vi "Stimulus.Open.vi"(8 "error in (no error)":errorcluster, 11 "State Variables":T1={"Events.State"=refnum, "Events.Test Result"=refnum, "Events.Progress"=refnum, "INI.Settings"={"Build Location"=path "C:/Simple Sequence Editor/SequenceRepo", "LoggingLocation"=path "", "Sequence.AbortChannel"="", "Sequence.IterationInfoChannel"="", "Sequence.DurationChannel"="", "Sequence.StepInfoChannel"="", "Sequence.SkipChannel"="", "PlotChannels"=[], "Sequence.InitializeScript"=path "C:/Simple Sequence Editor/SequenceRepo", "Sequence.CleanupScript"=path "", "Log.DefaultRate"=0.0}, "NIVS.AlarmManager"=refnum, "NIVS.BaseLogPath"=path "", "NIVS.DataLogManagerRef"=refnum, "NIVS.DataLogSpecRef"=refnum, "NIVS.Deployed"=FALSE, "NIVS.Events"={"SequenceEvent"=refnum, "SystemChangeEvent"=refnum, "WorkspaceEvent"=refnum}, "NIVS.GatewayIPAddress"="", "NIVS.DataLogGUID"="", "NIVS.ProfileCallback"=refnum, "NIVS.ProfileRef"=refnum, "NIVS.SequenceState"=enum."Idle", "NIVS.SystemDefinitionFile"=path "", "NIVS.SystemStateRefs"={"CustDatRef"=refnum, "EvtRef"=refnum, "Target State User Event"=refnum}, "NIVS.WorkspaceManager"=refnum, "NIVS.EventLogGUID"="", "NIVS.EventLogManagerRef"=refnum, "NIVS.EventLogSpecRef"=refnum, "NIVS.BaseToolPath"=path "", "Restart.Path"=path "", "Sequence.#ofColumns"=0, "Sequence.Iterations"=0, "Sequence.Channels"=[], "Sequence.ValidConfig?"=FALSE, "Station.ID"="", "UDP.Queue"=refnum, "UI.Abort"=refnum, "UI.Alarms"=refnum, "UI.Apply"=refnum, "UI.Back"=refnum, "UI.BaseFileName"=refnum, "UI.CurrentIteration"=refnum, "UI.CurrentStep"=refnum, "UI.CyclicFrequency"=refnum, "UI.Description"=refnum, "UI.DelayTime"=refnum, "UI.DisableAlarms"=refnum, "UI.Duration"=refnum, "UI.EnableLogging"=refnum, "UI.EnableState"=refnum, "UI.High"=refnum, "UI.LogChannels"=refnum, "UI.Low"=refnum, "UI.MonitoredVariable"=refnum, "UI.Next"=refnum, "UI.NumberOfCycles"=refnum, "UI.OperatorName"=refnum, "UI.Pause"=refnum, "UI.Profile"=refnum, "UI.Revert"=refnum, "UI.Skip"=refnum, "UI.Start"=refnum, "UI.StartIteration"=refnum, "UI.StartStep"=refnum, "UI.TabControl"=refnum, "UI.TotalIterations"=refnum, "UI.WaveformDefinition"=refnum, "UI.WaveformPreview"=refnum, "UI.WorkOrderNumber"=refnum, "UI.Chart"=refnum, "UI.Status"=refnum, "UI.DataView"=refnum, "UI.Table"=refnum, "UI.Multihead"=refnum, "UI.ToolTab"=refnum, "UI.Result"=refnum, "UI.Log Path"=refnum, "UI.ReportPath"=refnum, "UI.RestartPath"=refnum, "UI.AlarmLog"=refnum}) -> (0 "error out":errorcluster, 3 "State Variables":T1={"Events.State"=refnum, "Events.Test Result"=refnum, "Events.Progress"=refnum, "INI.Settings"={"Build Location"=path "C:/Simple Sequence Editor/SequenceRepo", "LoggingLocation"=path "", "Sequence.AbortChannel"="", "Sequence.IterationInfoChannel"="", "Sequence.DurationChannel"="", "Sequence.StepInfoChannel"="", "Sequence.SkipChannel"="", "PlotChannels"=[], "Sequence.InitializeScript"=path "C:/Simple Sequence Editor/SequenceRepo", "Sequence.CleanupScript"=path "", "Log.DefaultRate"=0.0}, "NIVS.AlarmManager"=refnum, "NIVS.BaseLogPath"=path "", "NIVS.DataLogManagerRef"=refnum, "NIVS.DataLogSpecRef"=refnum, "NIVS.Deployed"=FALSE, "NIVS.Events"={"SequenceEvent"=refnum, "SystemChangeEvent"=refnum, "WorkspaceEvent"=refnum}, "NIVS.GatewayIPAddress"="", "NIVS.DataLogGUID"="", "NIVS.ProfileCallback"=refnum, "NIVS.ProfileRef"=refnum, "NIVS.SequenceState"=enum."Idle", "NIVS.SystemDefinitionFile"=path "", "NIVS.SystemStateRefs"={"CustDatRef"=refnum, "EvtRef"=refnum, "Target State User Event"=refnum}, "NIVS.WorkspaceManager"=refnum, "NIVS.EventLogGUID"="", "NIVS.EventLogManagerRef"=refnum, "NIVS.EventLogSpecRef"=refnum, "NIVS.BaseToolPath"=path "", "Restart.Path"=path "", "Sequence.#ofColumns"=0, "Sequence.Iterations"=0, "Sequence.Channels"=[], "Sequence.ValidConfig?"=FALSE, "Station.ID"="", "UDP.Queue"=refnum, "UI.Abort"=refnum, "UI.Alarms"=refnum, "UI.Apply"=refnum, "UI.Back"=refnum, "UI.BaseFileName"=refnum, "UI.CurrentIteration"=refnum, "UI.CurrentStep"=refnum, "UI.CyclicFrequency"=refnum, "UI.Description"=refnum, "UI.DelayTime"=refnum, "UI.DisableAlarms"=refnum, "UI.Duration"=refnum, "UI.EnableLogging"=refnum, "UI.EnableState"=refnum, "UI.High"=refnum, "UI.LogChannels"=refnum, "UI.Low"=refnum, "UI.MonitoredVariable"=refnum, "UI.Next"=refnum, "UI.NumberOfCycles"=refnum, "UI.OperatorName"=refnum, "UI.Pause"=refnum, "UI.Profile"=refnum, "UI.Revert"=refnum, "UI.Skip"=refnum, "UI.Start"=refnum, "UI.StartIteration"=refnum, "UI.StartStep"=refnum, "UI.TabControl"=refnum, "UI.TotalIterations"=refnum, "UI.WaveformDefinition"=refnum, "UI.WaveformPreview"=refnum, "UI.WorkOrderNumber"=refnum, "UI.Chart"=refnum, "UI.Status"=refnum, "UI.DataView"=refnum, "UI.Table"=refnum, "UI.Multihead"=refnum, "UI.ToolTab"=refnum, "UI.Result"=refnum, "UI.Log Path"=refnum, "UI.ReportPath"=refnum, "UI.RestartPath"=refnum, "UI.AlarmLog"=refnum})   [LabVIEW 2015, in "Single Station Execution.lvlib"]
uses:
  Single Station Execution.lvlib
  Types/Main.StateVariables.ctl
  Types/INI.Settings.ctl
  <vilib>/NI Veristand/Execution/AlarmManager/AlarmManagerAPI.ctl
  NationalInstruments.VeriStand.ClientAPI
  <vilib>/NI Veristand/Execution/DataLogging/IDataLogging Ref.ctl
  <vilib>/NI Veristand/Execution/DataLogging/DataLoggingSpecification Ref.ctl
  Types/Execute.UserEventRefs.ctl
  <vilib>/NI Veristand/Execution/Workspace/SystemStateRegEventRef.ctl
  <vilib>/NI Veristand/Execution/Workspace/Target State Info.ctl
  <vilib>/NI Veristand/Execution/Workspace/Target State.ctl
  NationalInstruments.VeriStand.RealTimeSequenceDefinitionApi
  Types/Execution.SequenceState.ctl
  <vilib>/NI Veristand/Execution/Workspace/SystemStateEventRef.ctl
  <vilib>/NI Veristand/Execution/Workspace/WorkspaceAPI.ctl
  Types/UDPEngine.QueueCluster.ctl
  Types/UDPEngine.State.ctl
  <vilib>/NI Veristand/Execution/DataLogging/TDMS Property.ctl
  NationalInstruments.VeriStand.DataTypes
  <vilib>/NI Veristand/Execution/DataLogging/File Conflict Operation.ctl
  <vilib>/NI Veristand/Execution/DataLogging/Slope.ctl
  Main.Constants.vi
  <vilib>/NI Veristand/Execution/DataLogging/New Data Logging Specification (TDMS).vi
  <vilib>/NI Veristand/Execution/DataLogging/Set Data Logging Rate (Custom Rate).vi
  <vilib>/NI Veristand/Execution/DataLogging/Set Data Logging Rate (Target Rate).vi
  <vilib>/NI Veristand/Execution/DataLogging/Set Start Trigger (Start Immediately).vi
  <vilib>/NI Veristand/Execution/DataLogging/Set Start Trigger (Digital Edge).vi
  <vilib>/NI Veristand/Execution/DataLogging/Set Stop Trigger (Duration).vi
  <vilib>/NI Veristand/Execution/DataLogging/NI_VS Data Logging API.lvlib
  <vilib>/NI Veristand/Execution/Workspace/NI_VS Workspace ExecutionAPI.lvlib
  <vilib>/NI Veristand/Execution/AlarmManager/NI_VS AlarmManager ExecutionAPI.lvlib
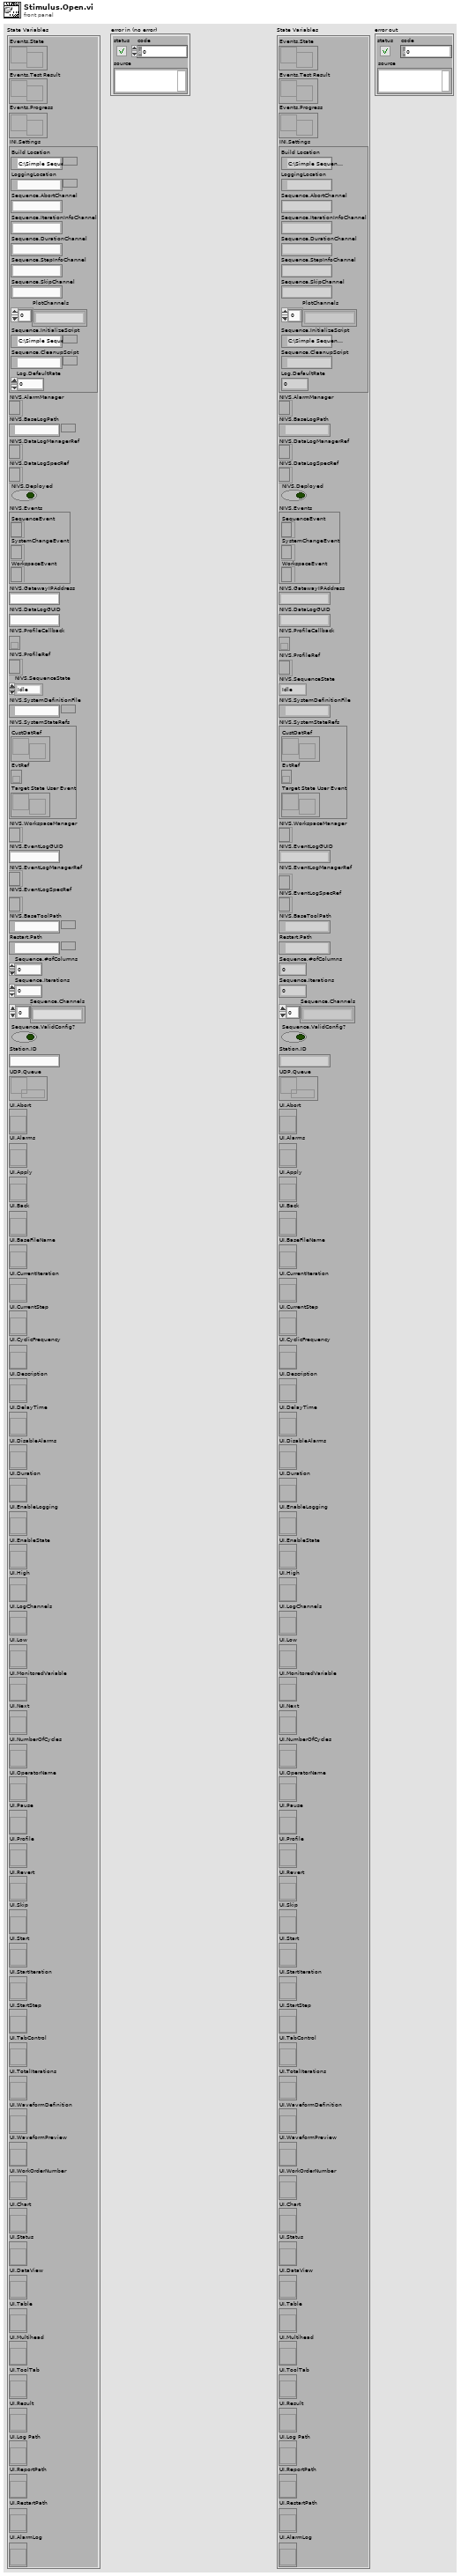
[diagram p1: front panel]
types:
  T1 = typedef "Single Station Execution.lvlib/Main.StateVariables.ctl" = cluster{"Events.State":refnum<user-event>, "Events.Test Result":refnum<user-event>, "Events.Progress":refnum<user-event>, "INI.Settings":T2, "NIVS.AlarmManager":T3, "NIVS.BaseLogPath":path, "NIVS.DataLogManagerRef":T4, "NIVS.DataLogSpecRef":T5, "NIVS.Deployed":bool, "NIVS.Events":T6, "NIVS.GatewayIPAddress":string, "NIVS.DataLogGUID":string, "NIVS.ProfileCallback":refnum<k27>, "NIVS.ProfileRef":refnum<k24>, "NIVS.SequenceState":T8, "NIVS.SystemDefinitionFile":path, "NIVS.SystemStateRefs":T9, "NIVS.WorkspaceManager":T10, "NIVS.EventLogGUID":string, "NIVS.EventLogManagerRef":T4, "NIVS.EventLogSpecRef":T5, "NIVS.BaseToolPath":path, "Restart.Path":path, "Sequence.#ofColumns":i32, "Sequence.Iterations":u32, "Sequence.Channels":string[], "Sequence.ValidConfig?":bool, "Station.ID":string, "UDP.Queue":refnum<queue>, "UI.Abort":refnum<vi>, "UI.Alarms":refnum<vi>, "UI.Apply":refnum<vi>, "UI.Back":refnum<vi>, "UI.BaseFileName":refnum<vi>, "UI.CurrentIteration":refnum<vi>, "UI.CurrentStep":refnum<vi>, "UI.CyclicFrequency":refnum<vi>, "UI.Description":refnum<vi>, "UI.DelayTime":refnum<vi>, "UI.DisableAlarms":refnum<vi>, "UI.Duration":refnum<vi>, "UI.EnableLogging":refnum<vi>, "UI.EnableState":refnum<vi>, "UI.High":refnum<vi>, "UI.LogChannels":refnum<vi>, "UI.Low":refnum<vi>, "UI.MonitoredVariable":refnum<vi>, "UI.Next":refnum<vi>, "UI.NumberOfCycles":refnum<vi>, "UI.OperatorName":refnum<vi>, "UI.Pause":refnum<vi>, "UI.Profile":refnum<vi>, "UI.Revert":refnum<vi>, "UI.Skip":refnum<vi>, "UI.Start":refnum<vi>, "UI.StartIteration":refnum<vi>, "UI.StartStep":refnum<vi>, "UI.TabControl":refnum<vi>, "UI.TotalIterations":refnum<vi>, "UI.WaveformDefinition":refnum<vi>, "UI.WaveformPreview":refnum<vi>, "UI.WorkOrderNumber":refnum<vi>, "UI.Chart":refnum<vi>, "UI.Status":refnum<vi>, "UI.DataView":refnum<vi>, "UI.Table":refnum<vi>, "UI.Multihead":refnum<vi>, "UI.ToolTab":refnum<vi>, "UI.Result":refnum<vi>, "UI.Log Path":refnum<vi>, "UI.ReportPath":refnum<vi>, "UI.RestartPath":refnum<vi>, "UI.AlarmLog":refnum<vi>}
  T2 = typedef "Single Station Execution.lvlib/INI.Settings.ctl" = cluster{"Build Location":path, "LoggingLocation":path, "Sequence.AbortChannel":string, "Sequence.IterationInfoChannel":string, "Sequence.DurationChannel":string, "Sequence.StepInfoChannel":string, "Sequence.SkipChannel":string, "PlotChannels":string[], "Sequence.InitializeScript":path, "Sequence.CleanupScript":path, "Log.DefaultRate":dbl}
  T3 = typedef "NI_VS AlarmManager ExecutionAPI.lvlib/AlarmManagerAPI.ctl" = refnum<k24>
  T4 = typedef "NI_VS Data Logging API.lvlib/IDataLogging Ref.ctl" = refnum<k24>
  T5 = typedef "NI_VS Data Logging API.lvlib/DataLoggingSpecification Ref.ctl" = refnum<k24>
  T6 = typedef "Single Station Execution.lvlib/Execute.UserEventRefs.ctl" = cluster{"SequenceEvent":refnum<event-registration>, "SystemChangeEvent":T7, "WorkspaceEvent":refnum<event-registration>}
  T7 = typedef "NI_VS Workspace ExecutionAPI.lvlib/SystemStateRegEventRef.ctl" = refnum<event-registration>
  T8 = typedef "Single Station Execution.lvlib/Execution.SequenceState.ctl" = enum16{"Idle", "Initializing", "Running", "Paused", "Finalizing", "Complete"}
  T9 = typedef "NI_VS Workspace ExecutionAPI.lvlib/SystemStateEventRef.ctl" = cluster{"CustDatRef":refnum<user-event>, "EvtRef":refnum<k27>, "Target State User Event":refnum<user-event>}
  T10 = typedef "NI_VS Workspace ExecutionAPI.lvlib/WorkspaceAPI.ctl" = refnum<k24>
  T11 = typedef "Single Station Execution.lvlib/Restart.Settings.ctl" = cluster{"LogFile":path, "Log Settings":T12[], "StimulusProfile":path, "StopIteration":u32, "StopStep":u32, "Log Channels":T16, "Base File Name":string, "Enable Logging":bool, "Profile":string, "StopDuration":dbl, "Waveform Definition":path, "Number of Cycles":dbl, "Cyclic Frequency":dbl, "Work Order Number":string, "Operator Name":string, "Description":string, "Station.ID":string, "Sequence.Channels":string[], "Alarms":T17[]}
  T12 = typedef "NI_VS Data Logging API.lvlib/TDMS Channel Group.ctl" = cluster{"Group Name":string, "Group Description":string, "Group Properties":T13[], "Channels":T14[], "Time Channel Options":T15, "Time Channel Name":string}
  T13 = typedef "NI_VS Data Logging API.lvlib/TDMS Property.ctl" = cluster{"Name":string, "Value":variant}
  T14 = typedef "NI_VS Data Logging API.lvlib/TDMS Channel.ctl" = cluster{"Channel Name":string, "Channel Path":string, "Channel Description":string, "Channel Properties":T13[]}
  T15 = typedef "NI_VS Data Logging API.lvlib/Time Channel Options.ctl" = enum16{"No Time Channel", "Absolute Time", "System Time", "System Time - Microseconds", "Absolute Time as Double", "Relative To First Start Trigger", "Relative To Session Start"}
  T16 = typedef "Single Station Execution.lvlib/Log.SelectedChannels.ctl" = enum16{"Channels (No System Channel)", "Aliases", "All"}
  T17 = typedef "Single Station Execution.lvlib/Config.AlarmSettings.ctl" = cluster{"Watch Channel":string, "High Limit":dbl, "Low Limit":dbl, "Delay":dbl, "State":enum16{"Disabled", "Enabled", "Tripped", "Delayed Trip", "Indicate"}, "Alarm Name":string}
  T18 = typedef "NI_VS Data Logging API.lvlib/File Conflict Operation.ctl" = enum16{"Create Unique", "Append to Existing", "Overwrite"}
  T19 = typedef "NI_VS Data Logging API.lvlib/Slope.ctl" = enum16{"Rising", "Falling"}
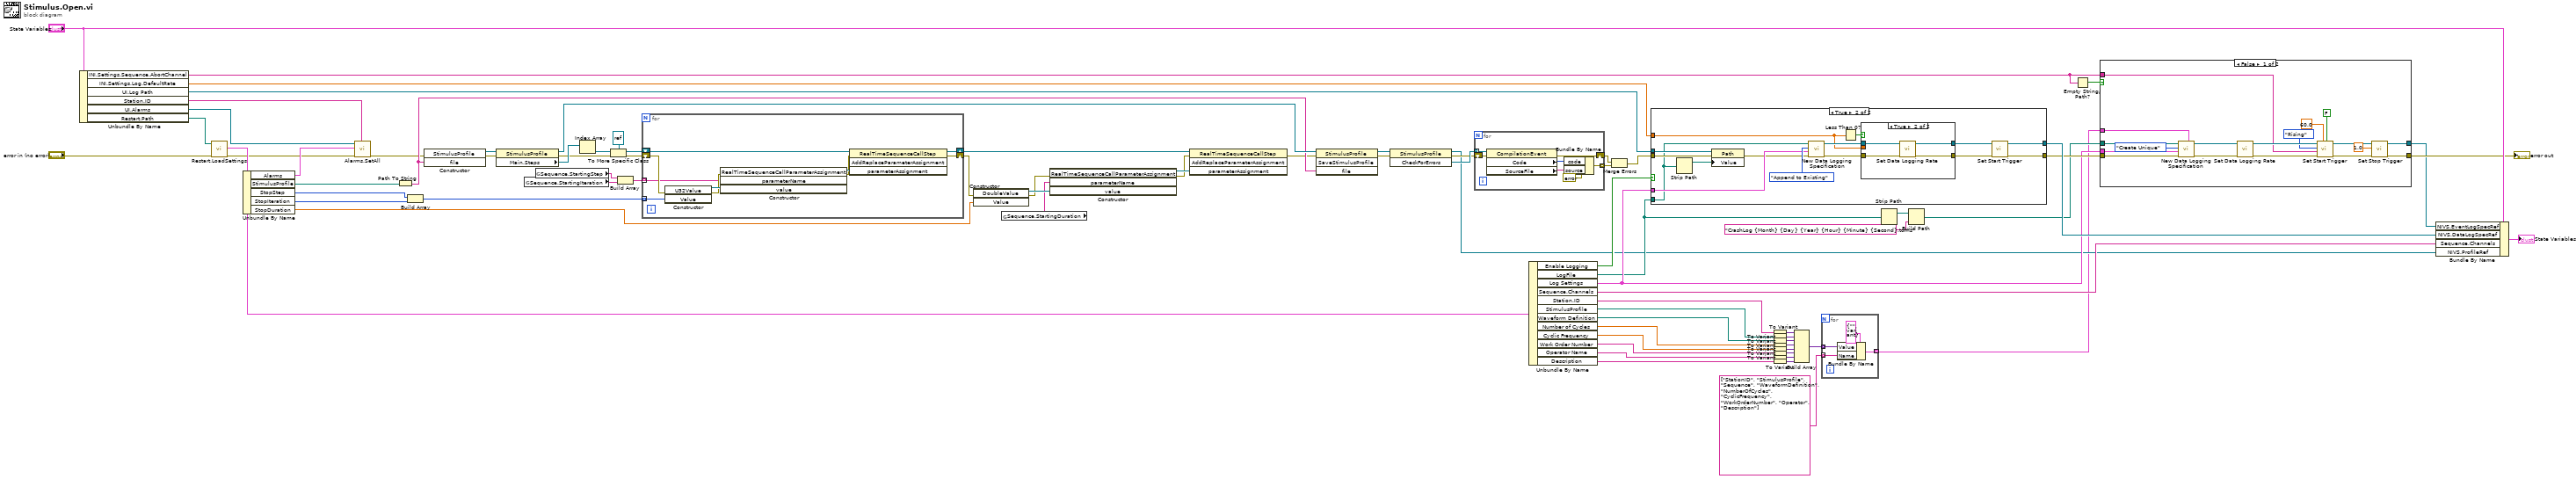
[diagram p0: block diagram]
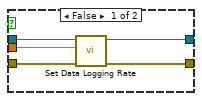
[diagram p4: hidden frame]
diagram:
  n1 = Unbundle By Name("State Variables") -> ("INI.Settings.Sequence.AbortChannel"=w25:string, "INI.Settings.Log.DefaultRate"=w37:dbl, "UI.Log Path"=w38:refnum<vi>, "Station.ID"=w1:string, "UI.Alarms"=w5:refnum<vi>, "Restart.Path"=w63:path)
  n2 = call "Restart.LoadSettings.vi"("error in"="error in (no error)", "path (use dialog)"=w63) -> ("error out"=w3:errorcluster, "Restart Settings"=w50:T11)  [unwired: 7 in, 1 out]
  n3 = Unbundle By Name(w50) -> ("Alarms"=w4:T17[], "StimulusProfile"=w60:path, "StopStep"=w61:u32, "StopIteration"=w62:u32, "StopDuration"=w41:dbl)
  n4 = call "Alarms.SetAll.vi"("Station.ID"=w1, "error in (no error)"=w3, "Alarms"=w4, "ListBox in"=w5) -> ("error out"=w2:errorcluster)  [unwired: 7 in]
  n5 = Path To String(path=w60) -> (string=w51:string)
  n6 = Build Array(w61, w62) -> (w53:u32[])
  n7 = constructor class="StimulusProfile"(error in=w2, "file"=w51) -> (reference out=w76:refnum<k24>, error out=w75:errorcluster)  [unwired: 2 in, 2 out]
  n8 = property class="StimulusProfile"(reference=w76, error in=w75) -> (reference out=w66:refnum<k24>, error out=w56:errorcluster, "Main.Steps"=w59:refnum<k24>[])
  n9 = global read "Main.Constants.vi" "Sequence.StartingIteration"() -> (w67:string)
  n10 = global read "Main.Constants.vi" "Sequence.StartingStep"() -> (w68:string)
  n11 = Index Array(array=w59) -> (element=w58:refnum<k24>)  [unwired: 1 in]
  n12 = To More Specific Class(target class=refnum<k24> refnum ("new reference"), reference=w58, error in=w56) -> (specific class reference=w55:refnum<k24>, error out=w52:errorcluster)
  n13 = Build Array(w68, w67) -> (w54:string[])
  n14 = for {
    tunnel: w54 -> [w81] mode=indexing
    tunnel: w53 -> [w79] mode=indexing
    shift-right: [w86] -> w42
    shift-left: w55 -> [w87]
    shift-right: [w88] -> w43
    shift-left: w52 -> [w82]
    n15 = constructor class="U32Value"(error in=w82, "Value"=w79) -> (reference out=w84:refnum<k24>, error out=w83:errorcluster)  [unwired: 2 in, 2 out]
    n16 = constructor class="RealTimeSequenceCallParameterAs"(error in=w83, "parameterName"=w81, "value"=w84) -> (reference out=w85:refnum<k24>, error out=w80:errorcluster)  [unwired: 2 in, 3 out]
    n17 = invoke class="RealTimeSequenceCallStep" method="AddReplaceParameterAssignment"(reference=w87, error in=w80, "parameterAssignment"=w85) -> (reference out=w86:refnum<k24>, error out=w88:errorcluster)  [unwired: 1 in, 2 out]
  }
  n18 = constructor class="DoubleValue"(error in=w43, "Value"=w41) -> (reference out=w47:refnum<k24>, error out=w46:errorcluster)  [unwired: 2 in, 2 out]
  n19 = global read "Main.Constants.vi" "Sequence.StartingDuration"() -> (w40:string)
  n20 = constructor class="RealTimeSequenceCallParameterAs"(error in=w46, "parameterName"=w40, "value"=w47) -> (reference out=w48:refnum<k24>, error out=w45:errorcluster)  [unwired: 2 in, 3 out]
  n21 = invoke class="RealTimeSequenceCallStep" method="AddReplaceParameterAssignment"(reference=w42, error in=w45, "parameterAssignment"=w48) -> (error out=w44:errorcluster)  [unwired: 1 in, 3 out]
  n22 = invoke class="StimulusProfile" method="SaveStimulusProfile"(reference=w66, error in=w44, "file"=w51) -> (reference out=w74:refnum<k24>, error out=w73:errorcluster)  [unwired: 1 in, 2 out]
  n23 = invoke class="StimulusProfile" method="CheckForErrors"(reference=w74, error in=w73) -> (reference out=w26:refnum<k24>, error out=w71:errorcluster, "CheckForErrors"=w72:refnum<k24>[])  [unwired: 1 in]
  n24 = for {
    tunnel: w72 -> [w95] mode=indexing
    tunnel: [w90] -> w69 mode=indexing
    shift-right: [w89] -> w70
    shift-left: w71 -> [w94]
    n25 = property class="CompilationEvent"(reference=w95, error in=w94) -> (error out=w89:errorcluster, "Code"=w92:i32, "SourceFile"=w91:string)  [unwired: 1 out]
    n26 = Bundle By Name(cluster=errorcluster {"status"=TRUE, "code"=0, "source"=""} ("error out"), "code"=w92, "source"=w91) -> (w90:errorcluster)
  }
  n27 = Unbundle By Name(w50) -> ("Enable Logging"=w27:bool, "LogFile"=w30:path, "Log Settings"=w33:T12[], "Sequence.Channels"=w39:string[], "Station.ID"=w7:string, "StimulusProfile"=w8:path, "Waveform Definition"=w9:path, "Number of Cycles"=w10:dbl, "Cyclic Frequency"=w11:dbl, "Work Order Number"=w12:string, "Operator Name"=w13:string, "Description"=w14:string)
  n28 = Merge Errors(w70, w69) -> (w49:errorcluster)
  n29 = case shown="True" w27 {
    tunnel: w49 -> [w96 w103]
    tunnel: [w96 w106] -> w35
    tunnel: [_ w105] -> w65
    tunnel: w30 -> [_ w97]
    tunnel: w33 -> [_ w104]
    tunnel: w38 -> [_ w101]
    tunnel: w37 -> [_ w99]
    frame False {
    }
    frame True {
      n30 = Strip Path(path=w97) -> (stripped path=w98:path)  [unwired: 1 out]
      n31 = property class="Path"(reference=w101, error in=w103, "Value"=w98) -> (error out=w102:errorcluster)  [unwired: 1 out]
      n32 = call-poly <vilib>:"New Data Logging Specification.vi"("error in (no error)"=w102, "Channel Groups"=w104, "File Conflict Operation"=File_Conflict_Operation."Append to Existing", "Base Log File Path"=w97) -> ("error out"=w108:errorcluster, "Data Logging Specification Ref out"=w111:T5)  [unwired: 6 in]
      n33 = Less Than 0?(x=w99) -> (x < 0?=w100:bool)
      n34 = case shown="True" w100 {
        tunnel: w111 -> [w116 w120]
        tunnel: [w113 w119] -> w110
        tunnel: [w114 w118] -> w109
        tunnel: w108 -> [w115 w117]
        tunnel: w99 -> [w112 _]
        frame False {
          n35 = call-poly <vilib>:"Set Data Logging Rate.vi"("error in (no error)"=w115, "Custom Rate (Hz)"=w112, "Data Logging Specification Ref in"=w116) -> ("error out"=w114:errorcluster, "Data Logging Specification Ref out"=w113:T5)  [unwired: 7 in]
        }
        frame True {
          n36 = call-poly <vilib>:"Set Data Logging Rate.vi"("error in (no error)"=w117, "Data Logging Specification Ref in"=w120) -> ("error out"=w118:errorcluster, "Data Logging Specification Ref out"=w119:T5)  [unwired: 8 in]
        }
      }
      n37 = call-poly <vilib>:"Set Start Trigger.vi"("error in (no error)"=w109, "Data Logging Specification Ref in"=w110) -> ("error out"=w106:errorcluster, "Data Logging Specification Ref out"=w105:T5)  [unwired: 8 in]
    }
  }
  n38 = To Variant(anything=w7) -> (Variant=w24:variant)
  n39 = To Variant(anything=w8) -> (Variant=w23:variant)
  n40 = To Variant(anything=w9) -> (Variant=w22:variant)
  n41 = To Variant(anything=w10) -> (Variant=w21:variant)
  n42 = To Variant(anything=w11) -> (Variant=w20:variant)
  n43 = To Variant(anything=w12) -> (Variant=w19:variant)
  n44 = To Variant(anything=w13) -> (Variant=w18:variant)
  n45 = To Variant(anything=w14) -> (Variant=w17:variant)
  n46 = Build Array(w24, w23, w22, w21, w20, w19, w18, w17) -> (w16:variant[])
  n47 = for {
    tunnel: w16 -> [w124] mode=indexing
    tunnel: string[] ["StationID", "StimulusProfile", "Sequence", "WaveformDefinition", "NumberOfCycles", "CyclicFrequency", "WorkOrderNumber", "Operator", "Description"] -> [w122] mode=indexing
    tunnel: [w121] -> w6 mode=indexing
    n48 = Bundle By Name(cluster=T13 {"Name"="", "Value"=variant} ("TDMS Property"), "Value"=w124, "Name"=w122) -> (w121:T13)
  }
  n49 = Strip Path(path=w30) -> (stripped path=w29:path)  [unwired: 1 out]
  n50 = Build Path(base path=w29, name or relative path="CrashLog {Month} {Day} {Year} {Hour} {Minute} {Second}.tdms") -> (appended path=w28:path)
  n51 = Empty String/Path?(string/path=w25) -> (empty?=w36:bool)
  n52 = case shown="False" w36 {
    tunnel: w35 -> [w130 w143]
    tunnel: [w127 w143] -> w34
    tunnel: w25 -> [w137 _]
    tunnel: [w126 _] -> w32
    tunnel: w33 -> [w129 _]
    tunnel: w28 -> [w128 _]
    tunnel: w6 -> [w125 _]
    frame False {
      n53 = call-poly <vilib>:"New Data Logging Specification.vi"("File Properties"=w125, "error in (no error)"=w130, "Channel Groups"=w129, "File Conflict Operation"=File_Conflict_Operation."Create Unique", "Base Log File Path"=w128) -> ("error out"=w141:errorcluster, "Data Logging Specification Ref out"=w138:T5)  [unwired: 5 in]
      n54 = call-poly <vilib>:"Set Data Logging Rate.vi"("error in (no error)"=w141, "Data Logging Specification Ref in"=w138) -> ("error out"=w140:errorcluster, "Data Logging Specification Ref out"=w139:T5)  [unwired: 8 in]
      n55 = call-poly <vilib>:"Set Start Trigger.vi"("Retriggerable (F)"=FALSE, "Pre-Trigger Duration (0 s)"=60.0, "error in (no error)"=w140, "Trigger Channel"=w137, "Slope"=Slope."Rising", "Data Logging Specification Ref in"=w139) -> ("error out"=w133:errorcluster, "Data Logging Specification Ref out"=w132:T5)  [unwired: 4 in]
      n56 = call-poly <vilib>:"Set Stop Trigger.vi"("error in (no error)"=w133, "Duration"=1.0, "Data Logging Specification Ref in"=w132) -> ("error out"=w127:errorcluster, "Data Logging Specification Ref out"=w126:T5)  [unwired: 7 in]
    }
    frame True {
    }
  }
  "error out" <- w34
  n57 = Bundle By Name(cluster="State Variables", "NIVS.EventLogSpecRef"=w32, "NIVS.DataLogSpecRef"=w65, "Sequence.Channels"=w39, "NIVS.ProfileRef"=w26) -> (→"State Variables":T1)
